vi "Coarse Frequency Synchronization.vi"(9 "Ts":dbl, 10 "Numeric in":dbl, 11 "Array in":cdb[](array[numeric])) -> (0 "Array out":cdb[](array[numeric]), 1 "coarse freq est":dbl)   [LabVIEW 2024]
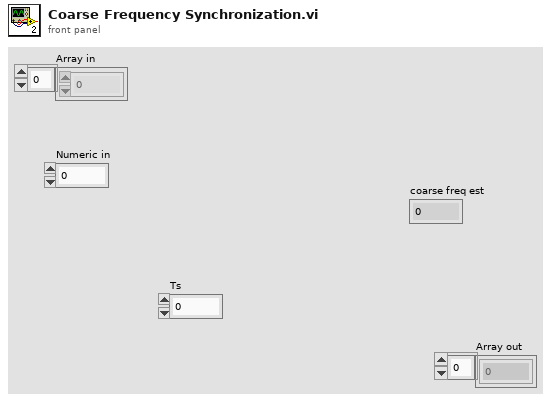
[diagram p1: front panel]
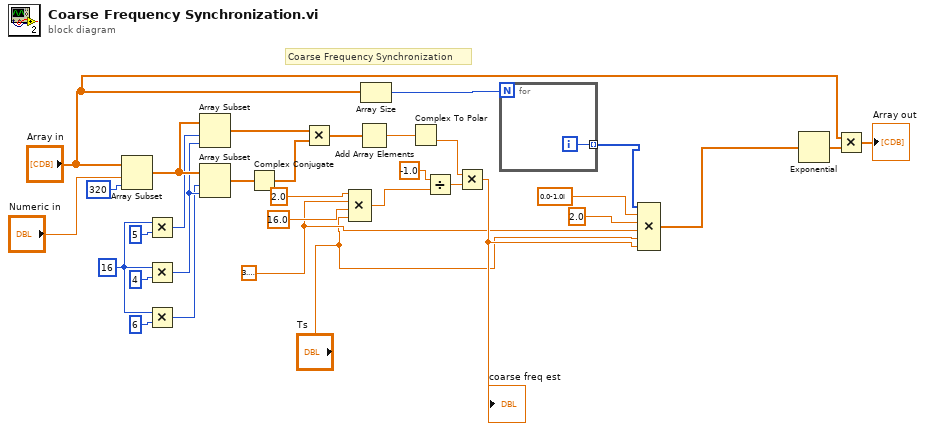
[diagram p0: block diagram]
diagram:
  w4 = 3.141592653589793
  w16 = 16 ("index")
  # "Coarse Frequency Synchronization"
  n1 = Array Subset(array="Array in", index="Numeric in", length=320) -> (w22:cdb[])
  n2 = Multiply(x=w16, y=5) -> (x*y=w14:i32)
  n3 = Multiply(x=w16, y=4) -> (x*y=w18:i32)
  n4 = Multiply(x=w16, y=6) -> (x*y=w15:i32)
  n5 = Array Subset(array=w22, index=w14, length=w18) -> (w27:cdb[])
  n6 = Array Subset(array=w22, index=w15, length=w18) -> (w19:cdb[])
  n7 = Complex Conjugate(1:w19) -> (0:w28:cdb[])
  n8 = Multiply(x=w27, y=w28) -> (x*y=w29:cdb[])
  n9 = Compound Arithmetic op=MULTIPLY(2.0 ("x"), w4, 16.0 ("x"), "Ts") -> (w10:dbl)
  n10 = Add Array Elements(numeric array=w29) -> (sum=w30:cdb)
  n11 = Array Size(array="Array in") -> (size(s)=w31:i32)
  n12 = Complex To Polar(r * e^(i*theta)=w30) -> (theta=w25:dbl)  [unwired: 1 out]
  n13 = Divide(x=-1.0, y=w10) -> (x/y=w21:dbl)
  n14 = Multiply ("Multiply.vi")(x=w25, y=w21) -> (x*y=w5:dbl)
  "coarse freq est" <- w5
  n15 = for {
    N: w31 -> [_]
    tunnel: [w33] -> w7 mode=indexing
    i -> [w33]
  }
  n16 = Compound Arithmetic op=MULTIPLY(w7, cdb 0.0-1.0i ("Real Matrix A"), 2.0 ("value"), w4, "Ts", w5) -> (w3:cdb[])
  n17 = Exponential ("Exponential.vi")(1:w3) -> (0:w23:cdb[])
  n18 = Multiply(x="Array in", y=w23) -> (x*y=→"Array out":cdb[])
